vi "write fd.vi"(4 "switch bitrate? (F)":bool, 5 "remote transmission request? (F)":bool, 6 "fd? (T)":bool=TRUE, 7 "extended id? (F)":bool, 8 "error in (no error)":errorcluster, 9 "data":u8[](array[numeric]) format="%x", 10 "id":u32 format="%x", 11 "channel handle":u16 format="%x") -> (0 "error out":errorcluster)   [LabVIEW 2024, in "atsj peakcan basic.lvlib"]
doc: "Writes a CAN FD message through an FD-capable PCAN bus (channel).\n\nCopyright (c) 2025 ATSJ (www.atsj.eu)"
uses:
  atsj peakcan basic.lvlib
  length 2 dlc.vi
  support/x64/PCANBasic.dll
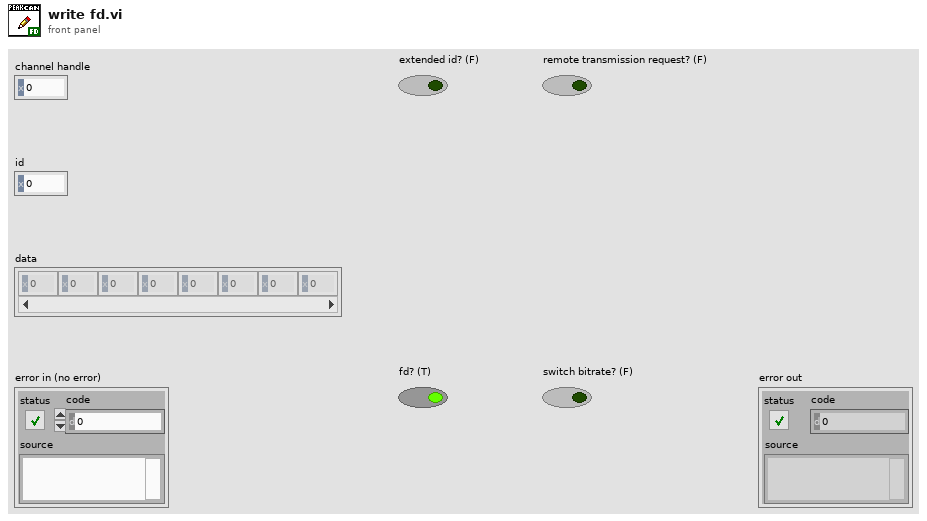
[diagram p1: front panel]
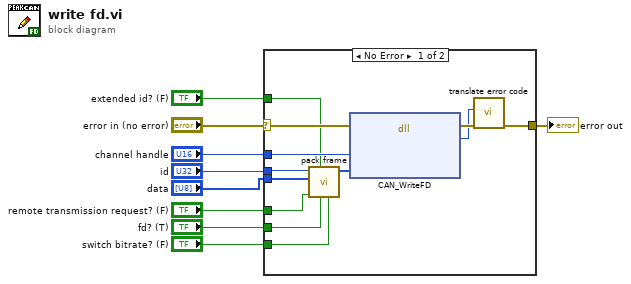
[diagram p0: block diagram]
diagram:
  n1 = case shown="No Error" "error in (no error)" {
    selector: "error in (no error)" -> [w17 w22]
    tunnel: "id" -> [w15 _]
    tunnel: "channel handle" -> [w21 _]
    tunnel: [w18 w22] -> w3
    tunnel: "data" -> [w14 _]
    tunnel: "extended id? (F)" -> [w13 _]
    tunnel: "remote transmission request? (F)" -> [w12 _]
    tunnel: "fd? (T)" -> [w11 _]
    tunnel: "switch bitrate? (F)" -> [w10 _]
    frame No Error {
      n2 = call "pack frame.vi"("switch bitrate? (F)"=w10, "can fd? (F)"=w11, "extended id?"=w13, "remote transmission request? (F)"=w12, "data"=w14, "id"=w15) -> ("frame"=w16:u8[])  [unwired: 5 in]
      n3 = dll-call lib="C:/atsj/plateau/atsj-peakcan-basic-for-labview/src/support/x64/PCANBasic.dll" fn="CAN_WriteFD"(error in=w17, "Channel"=w21, "MessageBuffer"=w16) -> (error out=w20:errorcluster, "Status"=w19:u32)  [unwired: 4 in, 1 out]
      n4 = call "translate error code.vi"("error in (no error)"=w20, "error code"=w19) -> ("error out"=w18:errorcluster)  [unwired: 9 in]
    }
    frame Error {
    }
  }
  "error out" <- w3
